vi "Test_Executor_Run_5.vi"(8 "error in":errorcluster, 10 "Wait ms":i32=2000, 11 "Sequence Path":path=path "C:/Users/DynaAdmin/PycharmProjects/Universal-sequence-executor-AF/configs/sequences/vtu_actual_sequence.json") -> (0 "error out":errorcluster)   [LabVIEW 2026]
doc: "Isolates Load: Load -> wait -> Normal Stop -> notify -> drain. Status shows the Load's own text (LOADED ... or LOAD ERROR: ...)."
uses:
  src/Executor/Sequence Executor.lvclass
  <vilib>/ActorFramework/Message Enqueuer/Message Enqueuer.lvclass/Message Enqueuer.ctl
  src/Executor Messages/Load Sequence Msg/Load Sequence Msg.lvclass/Load Sequence Msg.ctl
  <vilib>/ActorFramework/Message Enqueuer/Enqueue.vi
  <vilib>/ActorFramework/Stop Msg/Stop Msg.lvclass
  src/Executor Messages/Load Sequence Msg/Load Sequence Msg.lvclass
  <vilib>/ActorFramework/Message Priority Queue/Priority Enqueue.vi
  <vilib>/ActorFramework/Actor/Actor.lvclass
panel:
  out "Load error":errorcluster
  out "Stopped cleanly":bool
  out "Feedback Chart":dbl
  out "Verdict":string
  out "Channel Values":string[][](array[string])
  out "Step Table":string[][](array[string])
  out "Step Index":i32
  out "Status":string
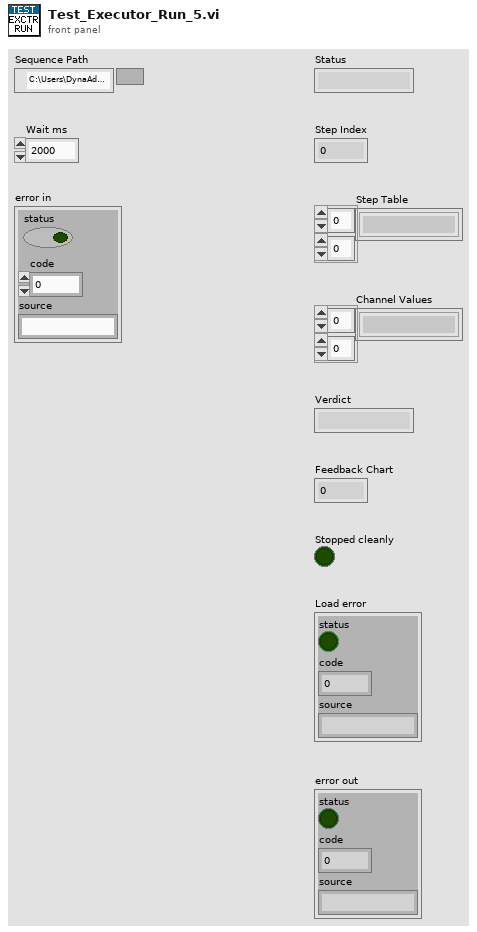
[diagram p1: front panel]
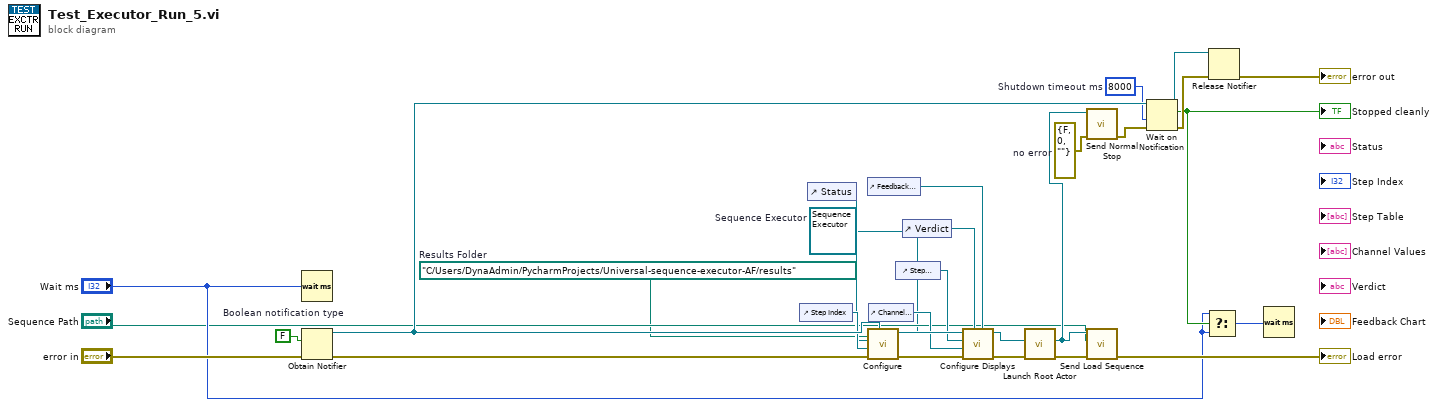
[diagram p0: block diagram]
diagram:
  w5 = path "C:/Users/DynaAdmin/PycharmProjects/Universal-sequence-executor-AF/results"  # Results Folder
  w4 = 8000  # Shutdown timeout ms
  w3 = errorcluster {"status"=FALSE, "code"=0, "source"=""}  # no error
  w2 = FALSE  # Boolean notification type
  w1 = refnum<class "Sequence Executor.lvclass"> refnum  # Sequence Executor
  n1 = Wait (ms)(milliseconds to wait="Wait ms") -> ()  [unwired: 1 out]
  n2 = Obtain Notifier(notification data type=w2, error in (no error)="error in") -> (notifier out=w15:refnum<notifier>, error out=w16:errorcluster)  [unwired: 2 in, 1 out]
  n3 = control-ref of="Step Index"() -> (w10:refnum<vi>)
  n4 = control-ref of="Status"() -> (w9:refnum<vi>)
  n5 = control-ref of="Feedback Chart"() -> (w14:refnum<vi>)
  n6 = call "Configure.vi"("Results Folder"=w5, "Stopped Notification"=w15, "error in"=w16, "Step Index Display"=w10, "Status Display"=w9, "Sequence Executor in"=w1) -> ("error out"=w18:errorcluster, "Sequence Executor out"=w17:refnum<class "Sequence Executor.lvclass">)  [unwired: 4 in]
  n7 = control-ref of="Channel Values"() -> (w12:refnum<vi>)
  n8 = control-ref of="Step Table"() -> (w11:refnum<vi>)
  n9 = control-ref of="Verdict"() -> (w13:refnum<vi>)
  n10 = call "Configure Displays.vi"("Feedback Chart"=w14, "Verdict Display"=w13, "error in"=w18, "Channel Values Display"=w12, "Step Table Display"=w11, "Sequence Executor in"=w17) -> ("error out"=w20:errorcluster, "Sequence Executor out"=w19:refnum<class "Sequence Executor.lvclass">)  [unwired: 4 in]
  n11 = call <vilib>:"Launch Root Actor.vi"("error in (no error)"=w20, "Actor"=w19) -> ("error out"=w22:errorcluster, "Actor's Enqueuer"=w21:refnum<class "Message Enqueuer.lvclass">)  [unwired: 8 in]
  n12 = call <vilib>:"Send Normal Stop.vi"("error in (no error)"=w3, "Message Enqueuer"=w21) -> ("error out"=w24:errorcluster)  [unwired: 9 in]
  n13 = call "Send Load Sequence.vi"("error in (no error)"=w22, "path"="Sequence Path", "Message Enqueuer"=w21) -> ("error out"=→"Load error":errorcluster)  [unwired: 7 in, 1 out]
  n14 = Wait on Notification(notifier=w15, timeout in ms (-1)=w4, error in (no error)=w24) -> (notifier out=w25:refnum<notifier>, notification=w26:bool, error out=w27:errorcluster)  [unwired: 1 in, 1 out]
  "Stopped cleanly" <- w26
  n15 = Select(t="Wait ms", s=w26, f="Wait ms") -> (s? t:f=w28:i32)
  n16 = Release Notifier(notifier=w25, error in (no error)=w27) -> (error out=→"error out":errorcluster)  [unwired: 1 in, 2 out]
  n17 = Wait (ms)(milliseconds to wait=w28) -> ()  [unwired: 1 out]
